vi "SC Get Tool Value.vi"(9 "tool lines":string[](array[string]), 10 "key":string) -> (1 "value":string, 2 "found?":bool)   [LabVIEW 2023]
doc: "Finds the last SYSTEMCORE-TOOL line that starts with key (e.g. ROBOT_DEPLOY) and returns the rest of the line."
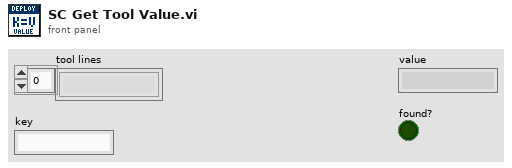
[diagram p1: front panel]
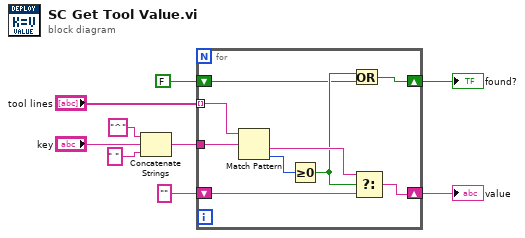
[diagram p0: block diagram]
diagram:
  n1 = Concatenate Strings("^", "key", " ") -> (w5:string)
  n2 = for {
    tunnel: "tool lines" -> [w18] mode=indexing
    tunnel: w5 -> [w17]
    shift-right: [w13] -> w4
    shift-left: "" -> [w14]
    shift-right: [w10] -> w2
    shift-left: FALSE -> [w11]
    n3 = Match Pattern(string=w18, regular expression=w17) -> (after substring=w15:string, offset past match=w16:i32)  [unwired: 1 in, 2 out]
    n4 = Greater Or Equal To 0?(x=w16) -> (x >= 0?=w12:bool)
    n5 = Or(x=w12, y=w11) -> (x .or. y?=w10:bool)
    n6 = Select(t=w15, s=w12, f=w14) -> (s? t:f=w13:string)
  }
  "value" <- w4
  "found?" <- w2
